vi "Get Dependency Paths.vi"(8 "error in (no error)":errorcluster, 11 "VI in":refnum<vi>) -> (0 "error out":errorcluster, 3 "DependencyPaths":path[](array[path]))   [LabVIEW 2019, in "Language Selection.lvlib"]
doc: "Get the Dependencies with the necessary options for the language toolkit.\n- - -\nCopyright (c) 2026, Merecs Engineering GmbH"
uses:
  Language Selection.lvlib
panel:
  out "spreadsheet string":string
  # "Connector Pane"
  # "Locals"
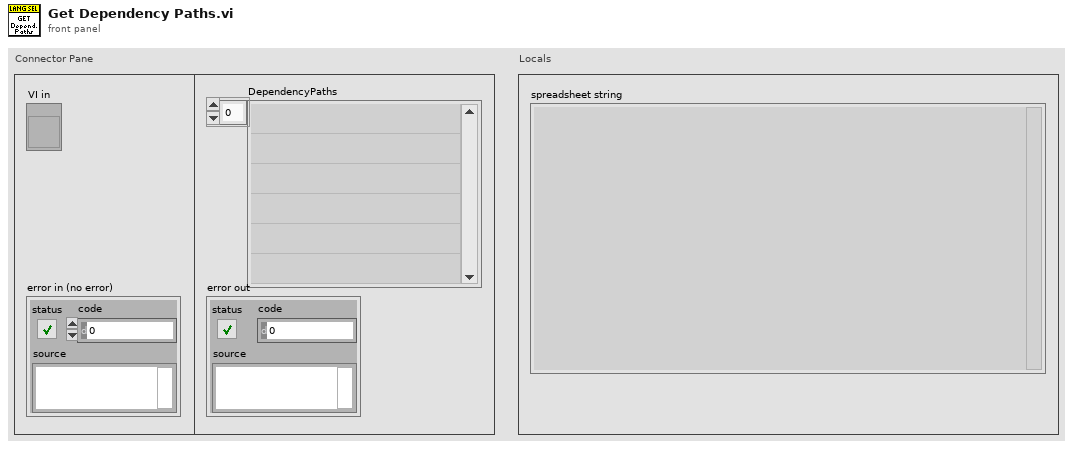
[diagram p1: front panel]
types:
  T1 = enum8{"No dynamic dispatch VIs", "Include nearest implementation", "Include all overrides"}
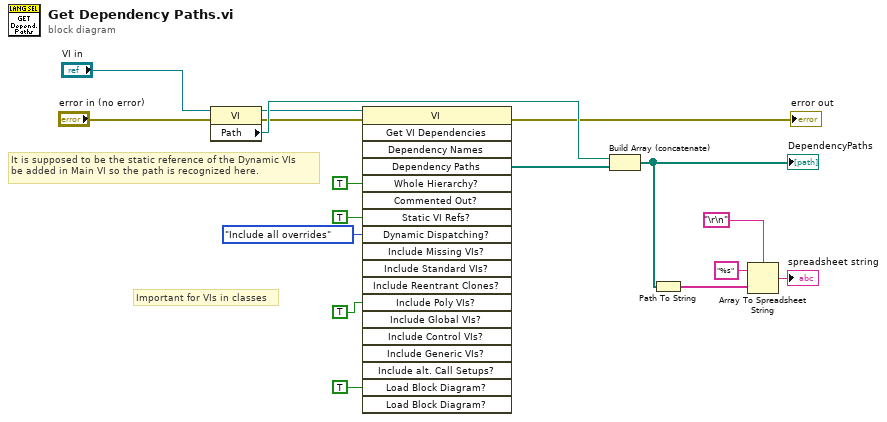
[diagram p0: block diagram]
diagram:
  # "Important for VIs in classes"
  # "It is supposed to be the static reference of the Dynamic VIs\nbe added in Main VI so the path is recognized here."
  n1 = property class="VI"(reference="VI in", error in="error in (no error)") -> (reference out=w8:refnum<vi>, error out=w10:errorcluster, "Path"=w15:path)
  n2 = invoke class="VI" method="Get VI Dependencies"(reference=w8, error in=w10, "Whole Hierarchy?"=TRUE, "Static VI Refs?"=TRUE, "Dynamic Dispatching?"=T1."Include all overrides", "Include Poly VIs?"=TRUE, "Load Block Diagram?"=TRUE ("Keep Express VIs?")) -> (error out=→"error out":errorcluster, "Dependency Paths"=w17:path[])  [unwired: 12 in, 17 out]
  n3 = Build Array (concatenate)(w15, w17) -> (w2:path[])
  "DependencyPaths" <- w2
  n4 = Path To String(path=w2) -> (string=w6:string[])
  n5 = Array To Spreadsheet String(delimiter (Tab)="\r\n", array=w6, 3:"%s" ("format string")) -> (spreadsheet string=→"spreadsheet string":string)
